vi "test tools call structured content.vi"(8 "error in (no error)":errorcluster) -> (0 "error out":errorcluster, 3 "body":string)   [LabVIEW 2020, in "MCP Server tests.lvlib"]
doc: "tools/call returns the outputs of a tool as structured content next to the text. fake_tool_picture_outputs has the outputs count (I32), label (string), time (timestamp), mode (enum) and picture (picture). Its result must carry structuredContent with exactly the four non-picture outputs, equal to the JSON object in the text item without the picture placeholder, and the picture must still arrive as an image item. A result with isError true has no structuredContent, both when the tool reports an error (fake_tool_return_error) and when a required argument is missing; an error cluster output that reports no error is an ordinary object in structuredContent. The requests are sent with the LabVIEW HTTP Client directly."
uses:
  MCP Server tests.lvlib
  bfb904d0-637c-4097-bbb0-3ed3f08b2a83.vi
  <vilib>/JDP Science/JSONtext/Next JSON Value.vi
  <vilib>/JDP Science/JSONtext/String Subset.vi
  <vilib>/JDP Science/JSONtext/Parsing/Advance past next JSON Value (inlined COPY).vi
  <vilib>/JDP Science/JSONtext/Parsing/Advance past whitespace.vi
  <vilib>/JDP Science/JSONtext/Parsing/Advance past String.vi
  <vilib>/JDP Science/JSONtext/Parsing/Advance past Number.vi
  <vilib>/JDP Science/JSONtext/Parsing/Advance past Line Ending.vi
  <vilib>/JDP Science/JSONtext/Parsing/Parse Full Path or Item Name.vi
  <vilib>/JDP Science/JSONtext/Parsing/Advance past Array.vi
  <vilib>/JDP Science/JSONtext/Parsing/Advance past Object.vi
  <vilib>/JDP Science/JSONtext/support/Error Cluster From Code.vi
  <vilib>/JDP Science/JSONtext/Offset/Find Item Locations by Path.vi
  <vilib>/JDP Science/JSONtext/support/Format JSON Object.vi
  <vilib>/JDP Science/JSONtext/JSON text to Variant.vi
  <vilib>/JDP Science/JSONtext/LVClass Serializer/JSONtext LVClass Serializer.lvclass
  <vilib>/addons/_JKI Toolkits/Caraya/classes/Test/Test.lvclass
  <vilib>/JDP Science/JSONtext/JSONtext.lvlib
  <vilib>/addons/_JKI Toolkits/Caraya/classes/Assert/Assert.lvclass
panel:
  out "lookup error":errorcluster
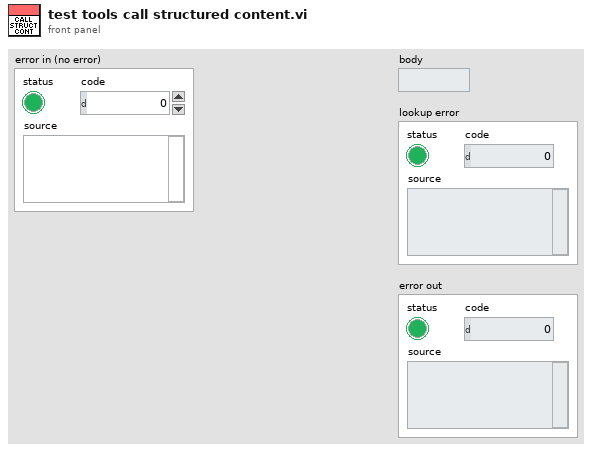
[diagram p1: front panel]
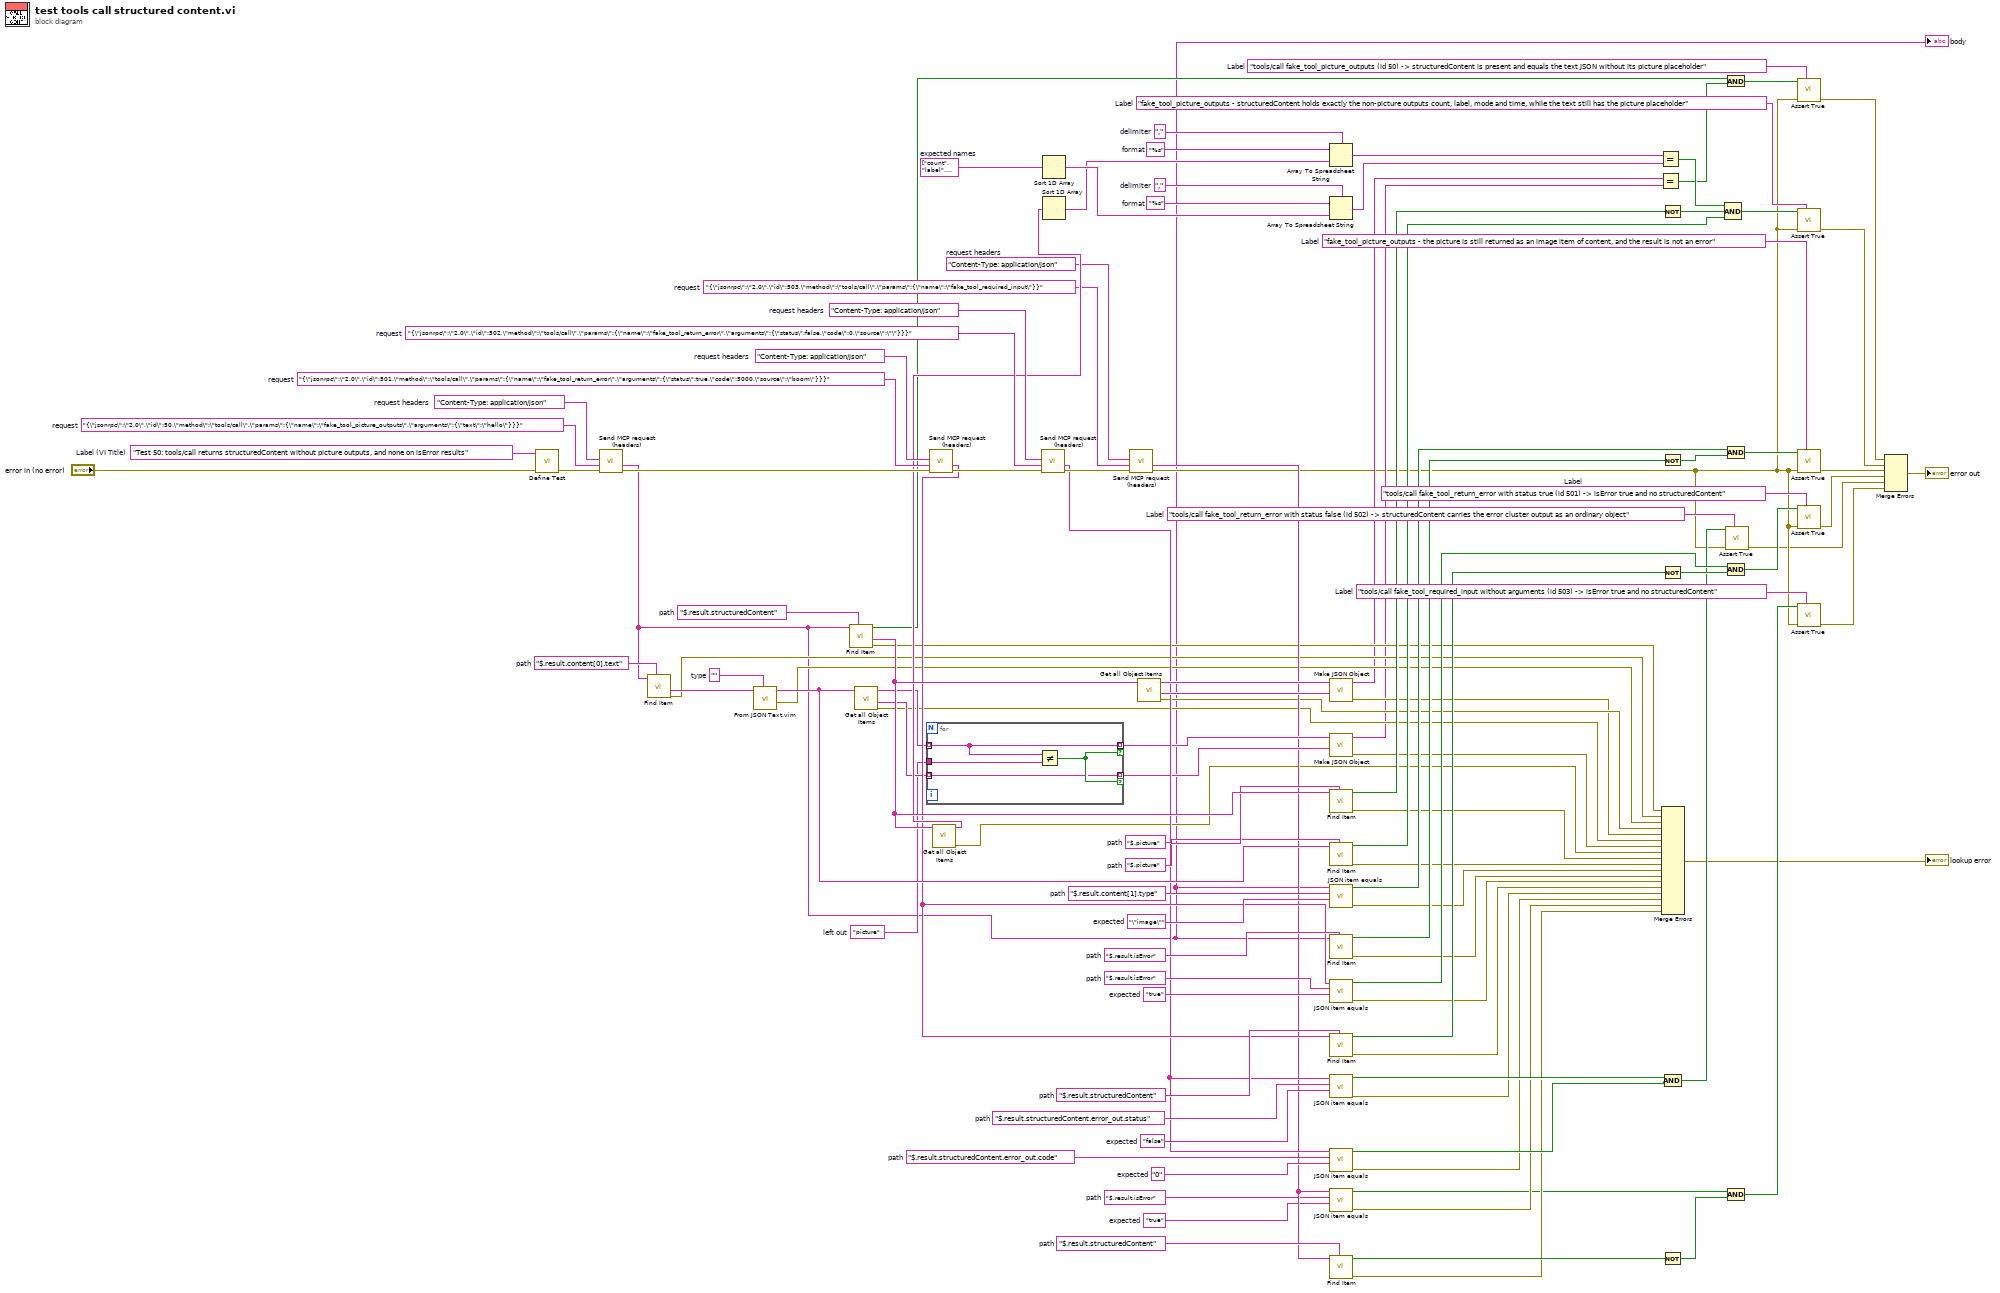
[diagram p0: block diagram]
diagram:
  w76 = "Content-Type: application/json"  # request headers
  w91 = "Content-Type: application/json"  # request headers
  w102 = "Content-Type: application/json"  # request headers
  w108 = "Content-Type: application/json"  # request headers
  w13 = "tools/call fake_tool_required_input without arguments (id 503) -> isError true and no structuredContent"  # Label
  w21 = "tools/call fake_tool_return_error with status false (id 502) -> structuredContent carries the error cluster output as an ordinary object"  # Label
  w46 = "tools/call fake_tool_return_error with status true (id 501) -> isError true and no structuredContent"  # Label
  w48 = "fake_tool_picture_outputs - the picture is still returned as an image item of content, and the result is not an error"  # Label
  w17 = "fake_tool_picture_outputs - structuredContent holds exactly the non-picture outputs count, label, mode and time, while the text still has the picture placeholder"  # Label
  w10 = "tools/call fake_tool_picture_outputs (id 50) -> structuredContent is present and equals the text JSON without its picture placeholder"  # Label
  w60 = "$.result.structuredContent"  # path
  w51 = "true"  # expected
  w52 = "$.result.isError"  # path
  w61 = "0"  # expected
  w62 = "$.result.structuredContent.error_out.code"  # path
  w64 = "false"  # expected
  w65 = "$.result.structuredContent.error_out.status"  # path
  w92 = "$.result.structuredContent"  # path
  w78 = "true"  # expected
  w79 = "$.result.isError"  # path
  w103 = "$.result.isError"  # path
  w94 = "\"image\""  # expected
  w95 = "$.result.content[1].type"  # path
  w83 = "$.picture"  # path
  w98 = "$.picture"  # path
  w109 = ","  # delimiter
  w111 = "%s"  # format
  w112 = string[] ["count", "label", "mode", "time"]  # expected names
  w71 = ","  # delimiter
  w73 = "%s"  # format
  w68 = "picture"  # left out
  w96 = ""  # type
  w104 = "$.result.content[0].text"  # path
  w105 = "$.result.structuredContent"  # path
  w75 = "{\"jsonrpc\":\"2.0\",\"id\":503,\"method\":\"tools/call\",\"params\":{\"name\":\"fake_tool_required_input\"}}"  # request
  w90 = "{\"jsonrpc\":\"2.0\",\"id\":502,\"method\":\"tools/call\",\"params\":{\"name\":\"fake_tool_return_error\",\"arguments\":{\"status\":false,\"code\":0,\"source\":\"\"}}}"  # request
  w101 = "{\"jsonrpc\":\"2.0\",\"id\":501,\"method\":\"tools/call\",\"params\":{\"name\":\"fake_tool_return_error\",\"arguments\":{\"status\":true,\"code\":5000,\"source\":\"boom\"}}}"  # request
  w107 = "{\"jsonrpc\":\"2.0\",\"id\":50,\"method\":\"tools/call\",\"params\":{\"name\":\"fake_tool_picture_outputs\",\"arguments\":{\"text\":\"hello\"}}}"  # request
  w114 = "Test 50: tools/call returns structuredContent without picture outputs, and none on isError results"  # Label (VI Title)
  n1 = call <vilib>:"Define Test.vi"("error in (no error)"="error in (no error)", "Label (VI Title)"=w114) -> ("error out"=w106:errorcluster)  [unwired: 8 in, 1 out]
  n2 = call "Send MCP request (headers).vi"("error in (no error)"=w106, "request"=w107, "request headers"=w108) -> ("error out"=w100:errorcluster, "response"=w3:string)  [unwired: 5 in, 2 out]
  "body" <- w3
  n3 = call <vilib>:"Find Item.vi"("$Path or Item Name"=w104, "JSON"=w3) -> ("error out"=w41:errorcluster, "<JSON>"=w97:string)  [unwired: 6 in, 2 out]
  n4 = call "From JSON Text.vim"("Data Type and Default Value"=w96, "JSON"=w97) -> ("error out"=w40:errorcluster, "Data out"=w84:string)  [unwired: 8 in]
  n5 = call <vilib>:"Find Item.vi"("$Path or Item Name"=w105, "JSON"=w3) -> ("error out"=w42:errorcluster, "<JSON>"=w99:string, "Found"=w16:bool)  [unwired: 6 in, 1 out]
  n6 = call <vilib>:"Get all Object Items.vi"("JSON"=w84) -> ("error out"=w37:errorcluster, "<JSON>"=w69:string[], "Item Names"=w70:string[])  [unwired: 7 in, 1 out]
  n7 = for {
    tunnel: w70 -> [w117] mode=indexing
    tunnel: w69 -> [w115] mode=indexing
    tunnel: w68 -> [w118]
    tunnel: [w117] -> w57 mode=indexing if=w116
    tunnel: [w115] -> w56 mode=indexing if=w116
    n8 = Not Equal?(x=w117, y=w118) -> (x != y?=w116:bool)
  }
  n9 = call "Send MCP request (headers).vi"("error in (no error)"=w100, "request"=w101, "request headers"=w102) -> ("error out"=w89:errorcluster, "response"=w80:string)  [unwired: 5 in, 2 out]
  n10 = call <vilib>:"Get all Object Items.vi"("JSON"=w99) -> ("error out"=w35:errorcluster, "Item Names"=w86:string[])  [unwired: 7 in, 2 out]
  n11 = call "Send MCP request (headers).vi"("error in (no error)"=w89, "request"=w90, "request headers"=w91) -> ("error out"=w74:errorcluster, "response"=w63:string)  [unwired: 5 in, 2 out]
  n12 = Sort 1D Array(array=w112) -> (sorted array=w110:string[])
  n13 = Sort 1D Array(array=w86) -> (sorted array=w72:string[])
  n14 = call "Send MCP request (headers).vi"("error in (no error)"=w74, "request"=w75, "request headers"=w76) -> ("error out"=w11:errorcluster, "response"=w53:string)  [unwired: 5 in, 2 out]
  n15 = call <vilib>:"Get all Object Items.vi"("JSON"=w99) -> ("error out"=w39:errorcluster, "<JSON>"=w87:string[], "Item Names"=w88:string[])  [unwired: 7 in, 1 out]
  n16 = Array To Spreadsheet String(delimiter (Tab)=w71, array=w72, 3:w73) -> (spreadsheet string=w59:string)
  n17 = Array To Spreadsheet String(delimiter (Tab)=w109, array=w110, 3:w111) -> (spreadsheet string=w58:string)
  n18 = call <vilib>:"Make JSON Object.vi"("JSON Items"=w87, "Item Names"=w88) -> ("error out"=w38:errorcluster, "<JSON>"=w24:string)  [unwired: 8 in]
  n19 = call <vilib>:"Make JSON Object.vi"("JSON Items"=w56, "Item Names"=w57) -> ("error out"=w36:errorcluster, "<JSON>"=w23:string)  [unwired: 8 in]
  n20 = call <vilib>:"Find Item.vi"("$Path or Item Name"=w98, "JSON"=w99) -> ("error out"=w34:errorcluster, "Found"=w85:bool)  [unwired: 6 in, 2 out]
  n21 = call <vilib>:"Find Item.vi"("$Path or Item Name"=w83, "JSON"=w84) -> ("error out"=w33:errorcluster, "Found"=w43:bool)  [unwired: 6 in, 2 out]
  n22 = call "JSON item equals.vi"("expected"=w94, "path"=w95, "JSON"=w3) -> ("error out"=w32:errorcluster, "equal?"=w82:bool)  [unwired: 6 in, 1 out]
  n23 = call <vilib>:"Find Item.vi"("$Path or Item Name"=w103, "JSON"=w3) -> ("error out"=w31:errorcluster, "Found"=w93:bool)  [unwired: 6 in, 2 out]
  n24 = call "JSON item equals.vi"("expected"=w78, "path"=w79, "JSON"=w80) -> ("error out"=w30:errorcluster, "equal?"=w67:bool)  [unwired: 6 in, 1 out]
  n25 = call <vilib>:"Find Item.vi"("$Path or Item Name"=w92, "JSON"=w80) -> ("error out"=w29:errorcluster, "Found"=w77:bool)  [unwired: 6 in, 2 out]
  n26 = call "JSON item equals.vi"("expected"=w64, "path"=w65, "JSON"=w63) -> ("error out"=w28:errorcluster, "equal?"=w55:bool)  [unwired: 6 in, 1 out]
  n27 = call "JSON item equals.vi"("expected"=w61, "path"=w62, "JSON"=w63) -> ("error out"=w27:errorcluster, "equal?"=w54:bool)  [unwired: 6 in, 1 out]
  n28 = call "JSON item equals.vi"("expected"=w51, "path"=w52, "JSON"=w53) -> ("error out"=w26:errorcluster, "equal?"=w20:bool)  [unwired: 6 in, 1 out]
  n29 = call <vilib>:"Find Item.vi"("$Path or Item Name"=w60, "JSON"=w53) -> ("error out"=w25:errorcluster, "Found"=w50:bool)  [unwired: 6 in, 2 out]
  n30 = Equal?(x=w59, y=w58) -> (x = y?=w45:bool)
  n31 = Equal?(x=w24, y=w23) -> (x = y?=w15:bool)
  n32 = Not(x=w85) -> (.not. x?=w44:bool)
  n33 = Not(x=w93) -> (.not. x?=w81:bool)
  n34 = Not(x=w77) -> (.not. x?=w66:bool)
  n35 = Not(x=w50) -> (.not. x?=w19:bool)
  n36 = Merge Errors(w42, w41, w40, w39, w38, w37, w36, w35, w34, w33, w32, w31, w30, w29, w28, w27, w26, w25) -> (→"lookup error":errorcluster)
  n37 = Compound Arithmetic op=AND(w55, w54) -> (w22:bool)
  n38 = Compound Arithmetic op=AND(w45, w44, w43) -> (w18:bool)
  n39 = call <vilib>:"Assert True.vi"("Label"=w21, "error in (no error)"=w11, "True?"=w22) -> ("error out"=w5:errorcluster)  [unwired: 7 in, 1 out]
  n40 = Compound Arithmetic op=AND(w16, w15) -> (w12:bool)
  n41 = Compound Arithmetic op=AND(w82, w81) -> (w49:bool)
  n42 = Compound Arithmetic op=AND(w67, w66) -> (w47:bool)
  n43 = Compound Arithmetic op=AND(w20, w19) -> (w14:bool)
  n44 = call <vilib>:"Assert True.vi"("Label"=w10, "error in (no error)"=w11, "True?"=w12) -> ("error out"=w9:errorcluster)  [unwired: 7 in, 1 out]
  n45 = call <vilib>:"Assert True.vi"("Label"=w17, "error in (no error)"=w11, "True?"=w18) -> ("error out"=w8:errorcluster)  [unwired: 7 in, 1 out]
  n46 = call <vilib>:"Assert True.vi"("Label"=w48, "error in (no error)"=w11, "True?"=w49) -> ("error out"=w7:errorcluster)  [unwired: 7 in, 1 out]
  n47 = call <vilib>:"Assert True.vi"("Label"=w46, "error in (no error)"=w11, "True?"=w47) -> ("error out"=w6:errorcluster)  [unwired: 7 in, 1 out]
  n48 = call <vilib>:"Assert True.vi"("Label"=w13, "error in (no error)"=w11, "True?"=w14) -> ("error out"=w4:errorcluster)  [unwired: 7 in, 1 out]
  n49 = Merge Errors(w9, w8, w7, w6, w5, w4) -> (→"error out":errorcluster)
